vi "Assign Help Info to VIs.vi"(5 "Save to Palettes (T)":bool=TRUE, 7 "Save to VIs (T)":bool=TRUE, 8 "error in":errorcluster, 10 "Source Files Help Info":T1(array[cluster]), 11 "Source File Paths":path[](array[path])) -> (0 "error out":errorcluster, 2 "dup Source Files Help Info":T1(array[cluster]), 3 "dup Source File Paths":path[](array[path]))   [LabVIEW 2014, in "VIHelpeksAPI.lvlib"]
doc: "The VI applies and saves the help linking information to the specified source VIs and palettes (.mnu files). Files other than VIs or palettes are ignored.\n\nThe <b>Example VI</b> demonstrating the use of VIHelpeks API can be opened using the \"Tools >> VI Helpeks >> Help and Support\" menu. Alternatively, you can launch the <b>NI Example Finder</b> and search for \"VI Helpeks\", or find it within the <b><labview>\\Examples\\VI Helpeks</b> folder.\n\n::: VI Helpeks :::\nCopyright (c) 2000-2026 Konstantin Shifershteyn. All rights reserved."
uses:
  VIHelpeksAPI.lvlib
  <vilib>/Palette API/Palette Menu/Public Type Define/Palette type.ctl
  <vilib>/Utility/lvfile.llb/NI_FileType.lvlib
  <vilib>/Palette API/Palette Menu/Palette Menu.lvlib
panel:
  # "VI Helpeks\nCopyright (c) 2012-2026 Konstantin Shifershteyn"
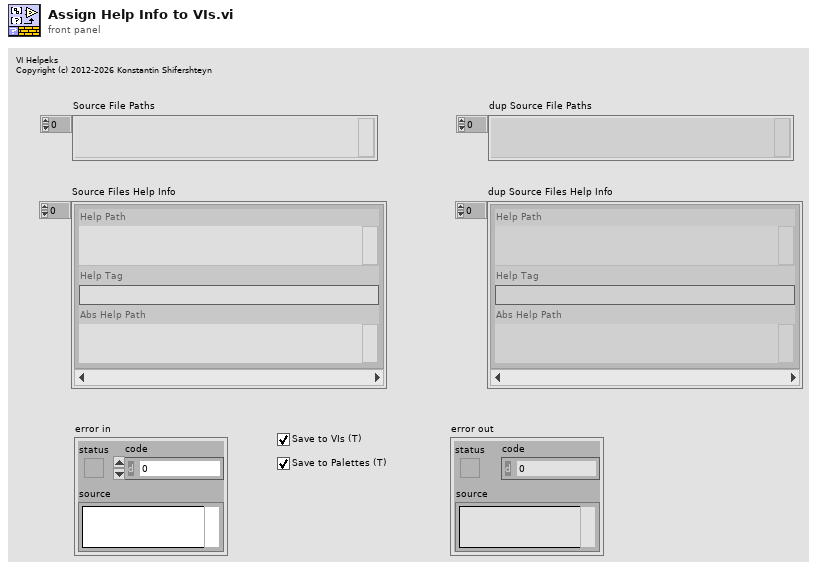
[diagram p1: front panel]
types:
  T1 = cluster{"Help Path":path, "Help Tag":string, "Abs Help Path":path}[]
  T2 = typedef "NI_FileType.lvlib/FT_FileTypes.ctl" = enum32{"Invalid file/path", "Unknown type", "Instrument", "Control", "Polymorphic VI", "Project", "Library", "LVClass", "XControl", "XNode", "CIN", "Run-time menu", "Palette menu", "LLB", "Shortcut", "Directory", "Class Private Data Control", "Statechart", "MathScript .m file", "Ladder Diagram", "LVLibp"}
  T3 = typedef "Palette Menu.lvlib/Palette type.ctl" = i32
  T4 = typedef "Palette Menu.lvlib/Palette Data.ctl" = cluster{"display name":string, "view format":T5, "palette width":i16, "items":T6, "256 color icon":picture, "B&W color icon":picture, "help information":T8, "palette description":string, "synchronize information":T9}
  T5 = typedef "Palette Menu.lvlib/View Format.ctl" = u16
  T6 = typedef "Palette Menu.lvlib/Items.ctl" = T7[]
  T7 = typedef "Palette Menu.lvlib/Item.ctl" = cluster{"item path":path, "library path (.lvlib)":path, "use default lvlib palette":bool, "short name":string, "place VI contents":bool, "hide synchronized item":bool, "reserve spot for synch item":bool, "configure when placing VI contents":bool}
  T8 = typedef "Palette Menu.lvlib/Help Info.ctl" = cluster{"help tag":string, "help file path ":path}
  T9 = typedef "Palette Menu.lvlib/Synchronize Info.ctl" = cluster{"synchronize with directory":bool, "synchronize directory path":path}
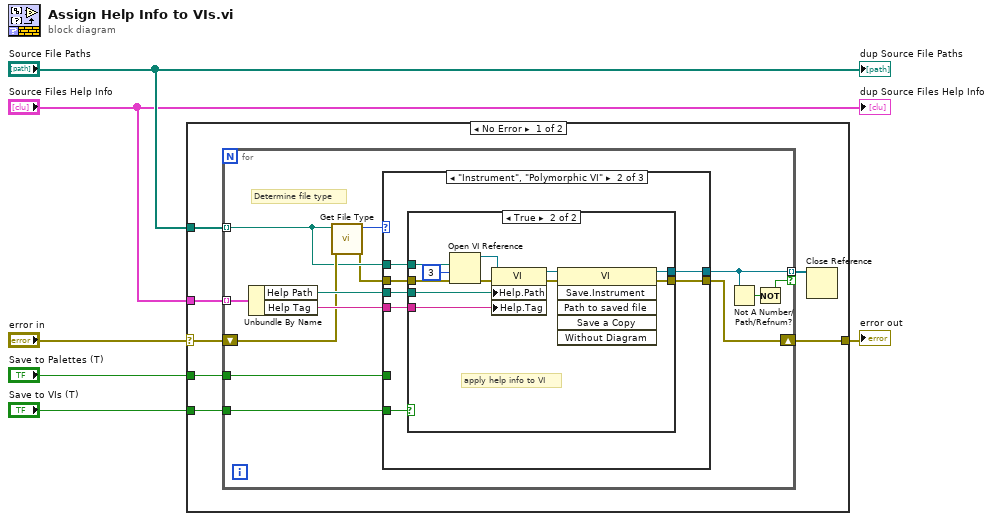
[diagram p0: block diagram]
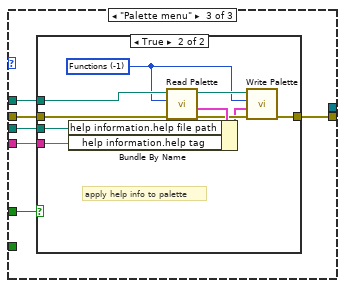
[diagram p4: hidden frame]
diagram:
  n1 = case shown="No Error" "error in" {
    selector: "error in" -> [w7 w64]
    tunnel: [w13 w64] -> w6
    tunnel: "Save to VIs (T)" -> [w12 _]
    tunnel: "Save to Palettes (T)" -> [w11 _]
    tunnel: "Source File Paths" -> [w10 _]
    tunnel: "Source Files Help Info" -> [w9 _]
    frame No Error {
      n2 = for {
        tunnel: w9 -> [w26] mode=indexing
        tunnel: [w16] -> w8 mode=indexing if=w14
        shift-right: [w22] -> w13
        shift-left: w7 -> [w21]
        tunnel: w10 -> [w20] mode=indexing
        tunnel: w12 -> [w18]
        tunnel: w11 -> [w17]
        # "Determine file type"
        n3 = Unbundle By Name(w26) -> ("Help Path"=w24:path, "Help Tag"=w23:string)
        n4 = call <vilib>:"Get File Type.vi"("error in (no error)"=w21, "path"=w20) -> ("error out"=w19:errorcluster, "file type"=w25:T2)  [unwired: 7 in, 1 out]
        n5 = case shown="\"Instrument\", \"Polymorphic VI\"" w25 {
          tunnel: w20 -> [_ w34 w51]
          tunnel: w24 -> [_ w33 w48]
          tunnel: w23 -> [_ w32 w49]
          tunnel: [_ w31 _] -> w16
          tunnel: w19 -> [w27 w29 w52]
          tunnel: [w27 w30 w50] -> w22
          tunnel: w18 -> [_ w28 _]
          tunnel: w17 -> [_ _ w47]
          frame Default {
          }
          frame "Instrument", "Polymorphic VI" {
            n6 = case shown="True" w28 {
              tunnel: w34 -> [_ w46]
              tunnel: w33 -> [_ w43]
              tunnel: w32 -> [_ w42]
              tunnel: [_ w40] -> w31
              tunnel: [w35 w38] -> w30
              tunnel: w29 -> [w35 w37]
              frame False {
              }
              frame True {
                # "apply help info to VI"
                n7 = Open VI Reference(vi path=w46, options=3, error in (no error)=w37) -> (vi reference=w44:refnum<vi>, error out=w45:errorcluster)  [unwired: 3 in]
                n8 = property class="VI"(reference=w44, error in=w45, "Help.Path"=w43, "Help.Tag"=w42) -> (reference out=w41:refnum<vi>, error out=w39:errorcluster)
                n9 = invoke class="VI" method="Save.Instrument"(reference=w41, error in=w39) -> (reference out=w40:refnum<vi>, error out=w38:errorcluster)  [unwired: 4 in, 4 out]
              }
            }
          }
          frame "Palette menu" {
            n10 = case shown="True" w47 {
              tunnel: w52 -> [w53 w63]
              tunnel: w51 -> [_ w62]
              tunnel: [w53 w56] -> w50
              tunnel: w49 -> [_ w55]
              tunnel: w48 -> [_ w54]
              frame False {
              }
              frame True {
                w59 = T3 -1 items=["Functions"=-1, "Controls"=-2] ("palette type")
                # "apply help info to palette"
                n11 = call <vilib>:"Read Palette.vi"("error in (no error)"=w63, "palette type"=w59, "palette path"=w62) -> ("error out"=w58:errorcluster, "palette data"=w61:T4, "duplicate palette path"=w60:path)  [unwired: 6 in]
                n12 = Bundle By Name(cluster=w61, "help information.help file path"=w54, "help information.help tag"=w55) -> (w57:T4)
                n13 = call <vilib>:"Write Palette.vi"("error in (no error)"=w58, "palette data"=w57, "palette type"=w59, "palette path"=w60) -> ("error out"=w56:errorcluster)  [unwired: 7 in]
              }
            }
          }
        }
        n14 = Not A Number/Path/Refnum?(number/path/refnum=w16) -> (NaN/Path/Refnum?=w15:bool)
        n15 = Not(x=w15) -> (.not. x?=w14:bool)
      }
      n16 = Close Reference(reference=w8) -> ()  [unwired: 1 in, 1 out]
    }
    frame Error {
    }
  }
  "error out" <- w6
  "dup Source File Paths" <- "Source File Paths"
  "dup Source Files Help Info" <- "Source Files Help Info"
